vi "PicoScope3000aExampleStreamingMSO.vi"() -> ()   [LabVIEW 2010]
doc: "This example demonstrates how to use the PicoScope Labview library to stream data from a PicoScope 5000 Series Device"
uses:
  ps3000a.dll
  ps3000aWrap.dll
  <vilib>/Waveform/DWDTOps.llb/DWDT Analog to Digital.vi
  PicoScope3000aLib/PicoScope3000aAnalogChannelSettings.ctl
  PicoScope3000aLib/PicoScope3000aDigitalChannelSettings.ctl
panel:
  in  "Port 0 Settings":T1={"Enabled"=FALSE, "Logic Level"=9830} {"Logic Level" items=["1.5V TTL"=9830, "2.5V CMOS"=16383]}
  in  "Trigger Settings":T2={"Trigger Enabled"=FALSE, "Trigger Source"=enum."Channel A", "Trigger Threshold (volts)"=0.0, "Trigger Direction"=2, "Trigger Delay (samples)"=0, "Auto Trigger Time (ms)"=1000} {"Trigger Direction" items=["Above", "Below", "Rising", "Falling", "Rising or Falling"]}
  in  "Channel A Settings":T3={"Enabled"=TRUE, "Coupling"=1, "Range"=6, "Analogue Offset"=0.0, "Bandwidth Limit"=0} {"Bandwidth Limit" items=["Full", "20MHz"]; "Range" items=["10 mV", "20 mV", "50 mV", "100 mV", "200 mV", "500 mV", "1 V", "2 V", "5 V", "10 V", "20 V", "50 V ", "100 V"]; "Coupling" items=["AC", "DC"]}
  out "Analog Channels":T4(graph)
  out "Raw Sample Interval (sec)":dbl=1.0000000130088963e-06 format="%#.5p"
  out "Max ADC value":i16
  out "Chunk time":u32
  out "Elapsed time":dbl
  in  "Poll time (ms)":u32=10 min=1 max=1000 step=1
  in  "Data file":path=path "PicoScope3000aExampleStreaming ChA Data"
  out "size(s)":i32
  out "Queue depth":i32(graph)
  out "queue depth":i32
  in  "Buffer and Transfer Settings":T5={"startIndex"=0, "Samples"=1000000, "Down Sample Ratio"=1, "Down-Sample Mode"=0} {"Down-Sample Mode" items=["None"=0, "Aggregate"=1, "Decimate"=2, "Average"=4]; "Down Sample Ratio" step=1; "Samples" format="%_6p"}
  out "USB Powered":bool=TRUE
  out "USB 3.0 device on non-USB 3.0 Port":bool=TRUE
  out "TriggeredAt (In Buffer)":u32 format="%#.6p"
  out "TriggeredAt (Total samples)":u32 format="%#.6p"
  in  "Acquisition Settings":T6={"Auto Stop"=TRUE, "Desired Sample Interval"=1, "Pre-trigger Samples"=0, "Post-trigger Samples"=1000000, "Down-Sample Ratio"=1, "Down-Sample Mode"=0, "Time Units"=3} {"Time Units" items=["Nanoseconds (ns)"=2, "Microseconds (us)"=3, "Milliseconds (ms)"=4, "Seconds (s)"=5]; "Down-Sample Mode" items=["None"=0, "Aggregate"=1, "Decimate"=2, "Average"=4]; "Post-trigger Samples" format="%#.6p"; "Pre-trigger Samples" format="%#_6p"}
  out "Port 0":digitalwaveform(graph)={"t0"=timestamp(0 s since 1904-01-01), "dt"=1.0000000130088963e-06, "Y"={"transitions"=[], "data"=[]}}
  out "Triggered":bool
  out "DownSample Interval (sec)":dbl=1.0000000130088963e-06 format="%#.5p"
  out "Total Samples":u32 format="%#.6p"
  out "Auto Stopped":bool
  in  "Serial Number":string
  in  "Open Using Serial Number":bool
  out "Number of Samples per Capture":u32 format="%#.6p"
  in  "Apply  Settings":bool
  in  "stop":bool
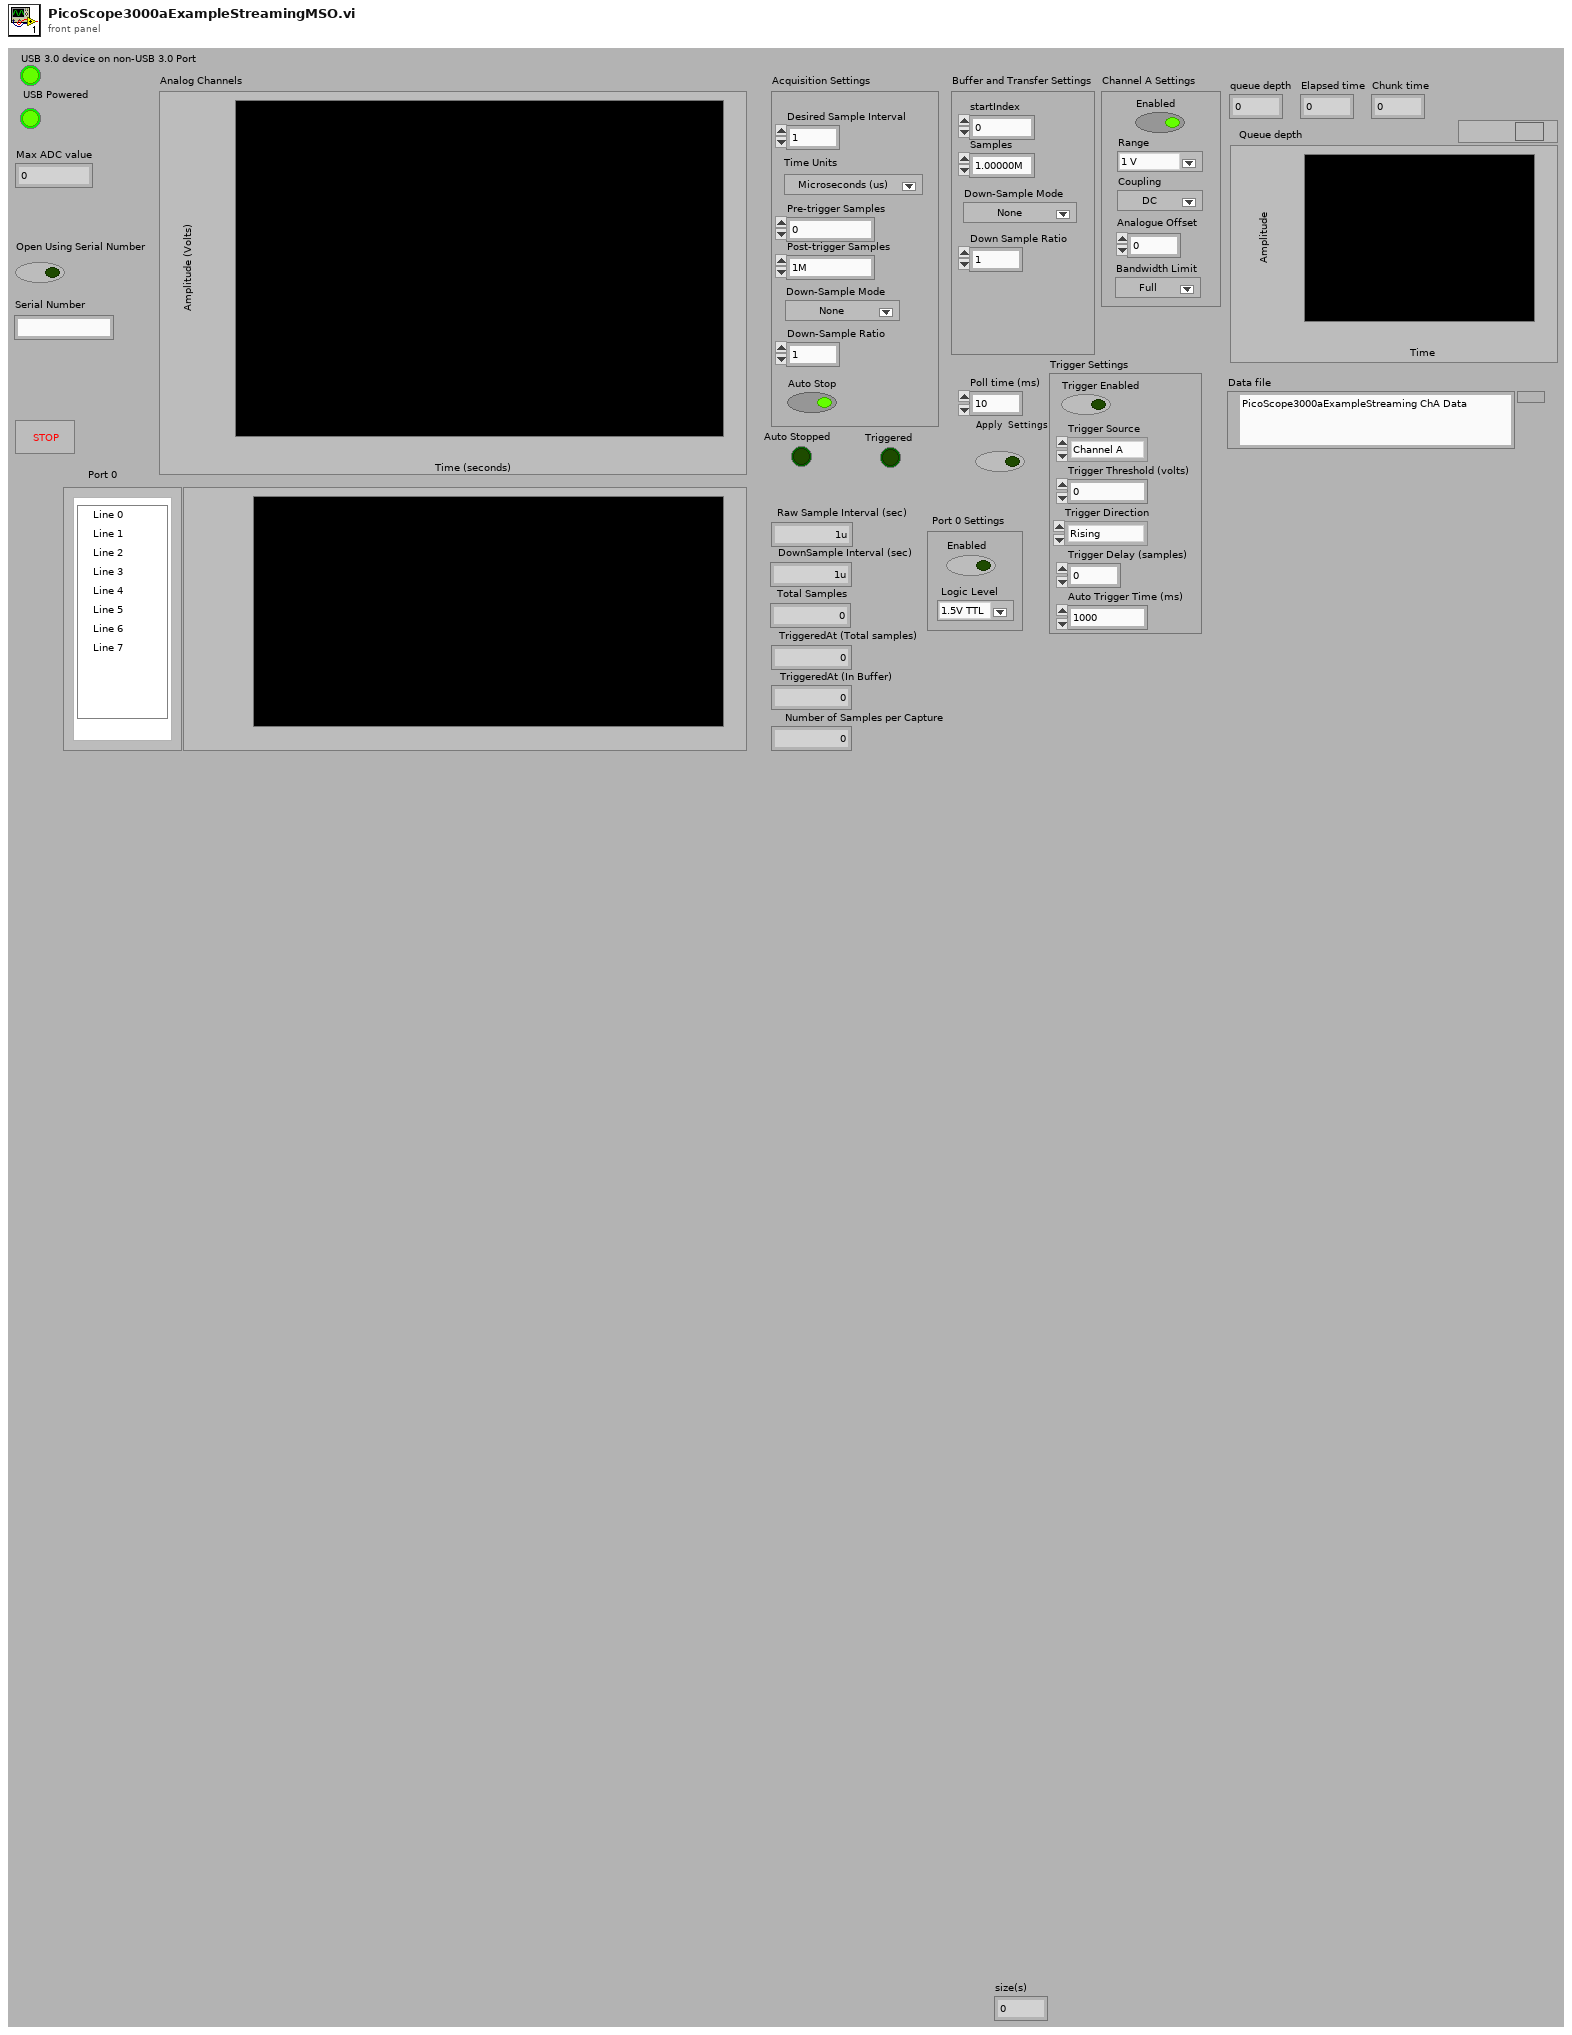
[diagram p1: front panel]
types:
  T1 = typedef "PicoScope3000aDigitalChannelSettings.ctl" = cluster{"Enabled":bool, "Logic Level":i16}
  T2 = cluster{"Trigger Enabled":bool, "Trigger Source":enum32{"Channel A", "Channel B", "Channel C", "Channel D", "Ext."}, "Trigger Threshold (volts)":dbl, "Trigger Direction":u32, "Trigger Delay (samples)":u32, "Auto Trigger Time (ms)":i16}
  T3 = typedef "PicoScope3000aAnalogChannelSettings.ctl" = cluster{"Enabled":bool, "Coupling":u32, "Range":u32, "Analogue Offset":sgl, "Bandwidth Limit":u32}
  T4 = cluster{i32, "DownSample Interval (sec)":dbl, "Data":dbl[]}
  T5 = cluster{"startIndex":u64, "Samples":u64, "Down Sample Ratio":u64, "Down-Sample Mode":u32}
  T6 = cluster{"Auto Stop":bool, "Desired Sample Interval":u32, "Pre-trigger Samples":u32, "Post-trigger Samples":u32, "Down-Sample Ratio":u32, "Down-Sample Mode":i32, "Time Units":u32}
  T7 = enum16{"open", "open or create", "create or replace", "create", "open (read-only)"}
  T8 = cluster{"Driver Version":string, "USB Version":string, "Hardware":string, "Variant":string, "Batch and Serial":string, "Cal Date":string, "Kernel Version":string, "Digital HW Version":string, "Analogue HW Version":string, "MSO":bool, "Number of channels":i16}
  T9 = cluster{"Channel A Buffer":i16[], "Channel B Buffer":i16[], "Channel C Buffer":i16[], "Channel D Buffer":i16[], "Channel E Buffer":i16[], "Channel F Buffer":i16[], "Channel G Buffer":i16[], "Channel H Buffer":i16[], "Port 0":i16[], "Port 1":i16[]}
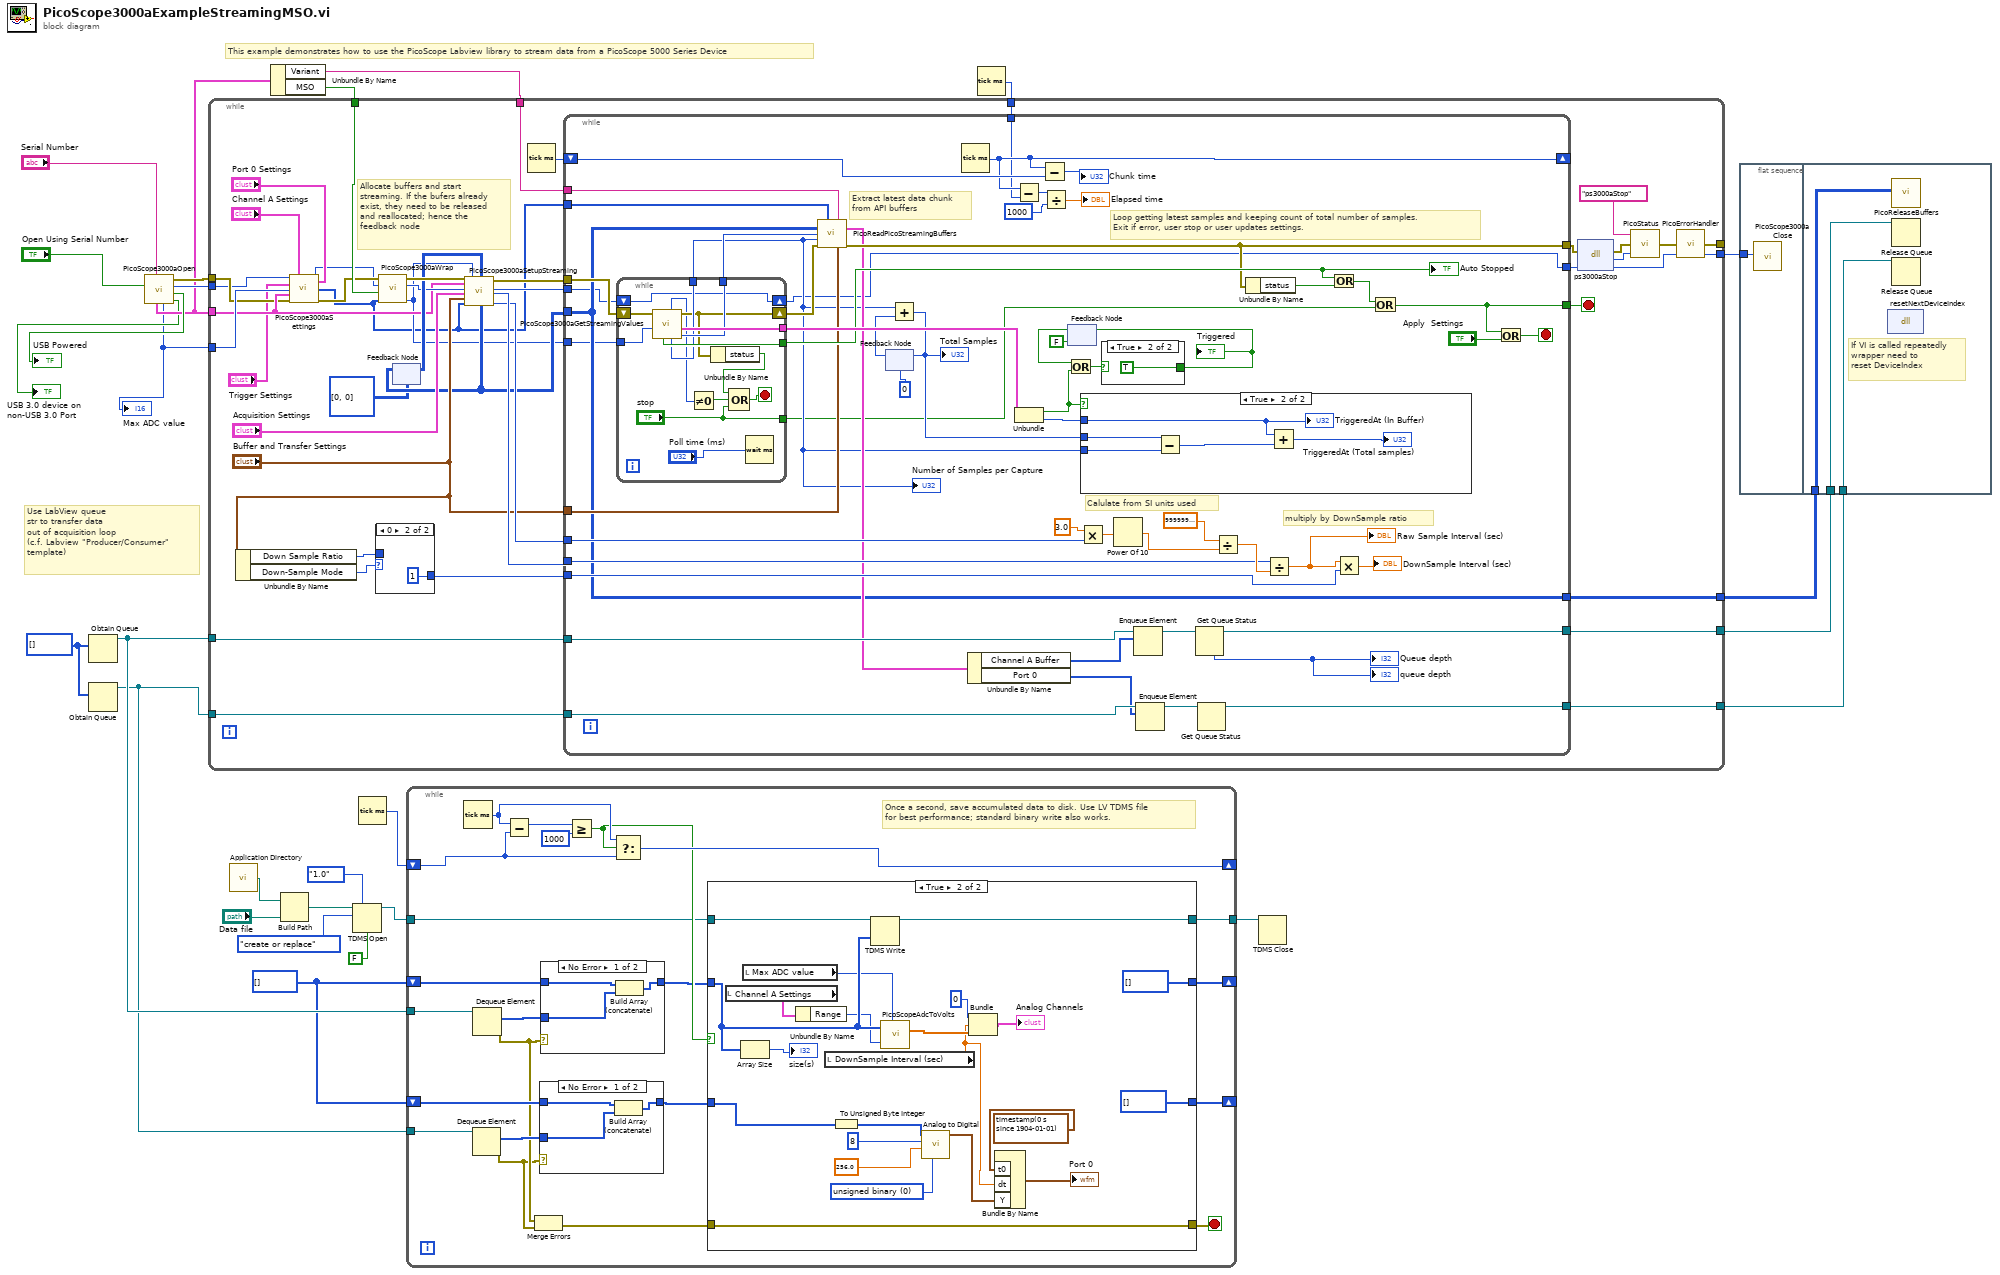
[diagram p0: block diagram]
diagram:
  w9 = i16[] [] ("History Data")
  w12 = i16[] [] ("History Data")
  # "Use LabView queue\nstr to transfer data\nout of acquisition loop\n(c.f. Labview \"Producer/Consumer\"\ntemplate)"
  # "This example demonstrates how to use the PicoScope Labview library to stream data from a PicoScope 5000 Series Device"
  n1 = Obtain Queue(element data type=w12) -> (queue out=w24:refnum<queue>)  [unwired: 4 in, 2 out]
  n2 = Obtain Queue(element data type=w12) -> (queue out=w10:refnum<queue>)  [unwired: 4 in, 2 out]
  n3 = call "PicoScope3000aOpen.vi"("Batch/Serial"="Serial Number", "Use Serial number"="Open Using Serial Number") -> ("USB 3.0 device on non-USB 3.0 Port"=→"USB 3.0 device on non-USB 3.0 Port":bool, "USB Powered"=→"USB Powered":bool, "handle"=w27:i16, "error out"=w28:errorcluster, "Max ADC value"=w1:i16, "Device Info"=w5:T8)  [unwired: 4 in]
  "Max ADC value" <- w1
  n4 = call <vilib>:"Application Directory.vi"() -> ("Application Directory"=w6:path)
  n5 = Unbundle By Name(w5) -> ("Variant"=w4:string, "MSO"=w3:bool)
  n6 = Build Path(base path=w6, name or relative path="Data file") -> (appended path=w7:path)
  n7 = TDMS Open(6:FALSE ("disable buffering? (T)"), 7:enum16{"1.0", "2.0"}."1.0" ("file format version (2.0)"), 10:T7."create or replace" ("operation (0:open)"), 11:w7) -> (3:w16:refnum<k34>)  [unwired: 2 in, 1 out]
  n8 = Tick Count (ms)() -> (millisecond timer value=w18:u32)
  n9 = while {
    tunnel: w24 -> [w49]
    shift-right: [w40] -> _
    shift-left: w9 -> [w48]
    shift-right: [w43] -> _
    shift-left: w18 -> [w44]
    tunnel: w16 -> [w39]
    tunnel: [w38] -> w15
    tunnel: w10 -> [w36]
    shift-right: [w33] -> _
    shift-left: w9 -> [w35]
    stop <- w29 stop-if-true
    # "Once a second, save accumulated data to disk. Use LV TDMS file\nfor best performance; standard binary write also works."
    n10 = Tick Count (ms)() -> (millisecond timer value=w45:u32)
    n11 = Dequeue Element(queue=w36) -> (element=w37:i16[], error out=w31:errorcluster)  [unwired: 2 in, 2 out]
    n12 = Dequeue Element(queue=w49) -> (element=w50:i16[], error out=w32:errorcluster)  [unwired: 2 in, 2 out]
    n13 = Subtract(x=w45, y=w44) -> (x-y=w47:u32)
    n14 = Merge Errors(w32, w31) -> (w30:errorcluster)
    n15 = case shown="No Error" w31 {
      tunnel: w35 -> [w53 w54]
      tunnel: [w52 w54] -> w34
      tunnel: w37 -> [w51 _]
      frame No Error {
        n16 = Build Array (concatenate)(w53, w51) -> (w52:i16[])
      }
      frame Error {
      }
    }
    n17 = case shown="No Error" w32 {
      tunnel: w48 -> [w83 w84]
      tunnel: [w82 w84] -> w41
      tunnel: w50 -> [w81 _]
      frame No Error {
        n18 = Build Array (concatenate)(w83, w81) -> (w82:i16[])
      }
      frame Error {
      }
    }
    n19 = Greater Or Equal?(x=w47, y=u32 1000) -> (x >= y?=w42:bool)
    n20 = Select(t=w45, s=w42, f=w44) -> (s? t:f=w43:u32)
    n21 = case shown="True" w42 {
      tunnel: w41 -> [w58 w76]
      tunnel: [w58 i16[] [] ("History Data")] -> w40
      tunnel: w39 -> [w57 w78]
      tunnel: [w57 w77] -> w38
      tunnel: w34 -> [w56 w63]
      tunnel: [w56 i16[] [] ("History Data")] -> w33
      tunnel: w30 -> [w55 w59]
      tunnel: [w55 w59] -> w29
      frame False {
      }
      frame True {
        w69 = u16 0 items=["unsigned binary", "offset binary", "2's complement"] ("data format (offset binary)")
        n22 = local read "Channel A Settings"() -> (w60:T3)
        n23 = Array Size(array=w76) -> (size(s)=→"size(s)":i32)
        n24 = local read "Max ADC value"() -> (w72:i16)
        n25 = Unbundle By Name(w60) -> ("Range"=w75:u32)
        n26 = local read "DownSample Interval (sec)"() -> (w64:dbl)
        n27 = To Unsigned Byte Integer(number=w63) -> (unsigned 8bit integer=w68:u8[])
        n28 = TDMS Write(0:w78, 9:w76) -> (4:w77:refnum<k34>)  [unwired: 4 in, 3 out]
        n29 = call "PicoScopeAdcToVolts.vi"("Max_adc"=w72, "Range Index"=w75, "Data"=w76) -> ("Data"=w73:dbl[])
        n30 = call-poly <vilib>:"Analog to Digital.vi"("data format (offset binary)"=w69, "full-scale range (pk-pk)"=256.0, "resolution (16 bit)"=8, "analog waveform"=w68) -> ("digital waveform"=w65:digitalwaveform)  [unwired: 4 in, 3 out]
        n31 = Bundle(0, "DownSample Interval (sec)"=w64, "Data"=w73) -> (→"Analog Channels":T4)  [unwired: 1 in]
        n32 = Bundle By Name("t0"=timestamp(0 s since 1904-01-01), "dt"=w64, "Y"=w65) -> (→"Port 0":digitalwaveform)  [unwired: 1 in]
      }
    }
  }
  n33 = Tick Count (ms)() -> (millisecond timer value=w23:u32)
  n34 = while {
    tunnel: [w123] -> w22
    tunnel: w28 -> [w90]
    tunnel: w27 -> [w89]
    tunnel: w5 -> [w92]
    tunnel: w1 -> [w95]
    tunnel: [w109] -> w20
    tunnel: w24 -> [w108]
    tunnel: [w107] -> w21
    tunnel: [w105] -> _
    tunnel: w23 -> [w103]
    tunnel: [w100] -> w11
    tunnel: w10 -> [w99]
    tunnel: w4 -> [w98]
    tunnel: w3 -> [w96]
    stop <- w127 stop-if-true
    # "Allocate buffers and start\nstreaming. If the bufers already\nexist, they need to be released\nand reallocated; hence the\nfeedback node"
    n35 = Unbundle By Name("Buffer and Transfer Settings") -> ("Down Sample Ratio"=w112:u64, "Down-Sample Mode"=w114:u32)
    n36 = call "PicoScope3000aSettings.vi"("handle in"=w89, "Channel A Settings"="Channel A Settings", "Port 0 Settings"="Port 0 Settings", "Trigger Settings"="Trigger Settings", "Max_adc"=w95, "Device Info"=w92, "error in"=w90) -> ("handle out"=w86:i16, "Enabled Array"=w85:i16[], "error out"=w87:errorcluster)  [unwired: 6 in]
    n37 = case shown="0" w114 {
      tunnel: [w128 u32 1 ("Down-Sample Ratio")] -> w113
      tunnel: w112 -> [w128 _]
      frame Default {
      }
      frame 0 {
      }
    }
    n38 = call "PicoScope3000aWrap.vi"("Enabled Array"=w85, "MSO Device?"=w96, "handle in"=w86, "error in (no error)"=w87) -> ("deviceIndex"=w91:u16, "handle out"=w93:i16, "error out"=w118:errorcluster)  [unwired: 1 in]
    n39 = feedback #1(u64[][] [[0], [0]] ("Pointer array")) -> (w106:u64[][])
    n40 = call "PicoScope3000aSetupStreaming.vi"("error in"=w118, "Device Info"=w92, "handle in"=w93, "Acquisition Settings"="Acquisition Settings", "Buffer and Transfer Settings"="Buffer and Transfer Settings", "enabled array"=w85, "deviceIndex"=w91, "Pointers In"=w106) -> ("Pointer array"=w102:u64[][], "error out"=w125:errorcluster, "handle out"=w126:i16, "Sample Interval"=w117:u32, "sampleIntervalTimeUnits"=w116:u32)  [unwired: 7 in]
    n41 = feedback-in #1(w102) -> ()
    n42 = Tick Count (ms)() -> (millisecond timer value=w104:u32)
    n43 = while {
      tunnel: [w130] -> w124
      tunnel: [w184] -> w127
      tunnel: w126 -> [w131]
      tunnel: w125 -> [w160]
      tunnel: w117 -> [w163]
      tunnel: w116 -> [w171]
      tunnel: [w157] -> w115
      tunnel: w113 -> [w161]
      tunnel: "Buffer and Transfer Settings" -> [w159]
      tunnel: w85 -> [w156]
      tunnel: [w154] -> w109
      tunnel: w108 -> [w152]
      tunnel: w102 -> [w150]
      tunnel: [w150] -> w107
      shift-right: [w145] -> _
      shift-left: w104 -> [w146]
      tunnel: w103 -> [w144]
      tunnel: w98 -> [w139]
      tunnel: [w136] -> w100
      tunnel: w99 -> [w135]
      tunnel: w91 -> [w132]
      stop <- w183 stop-if-true
      # "Loop getting latest samples and keeping count of total number of samples. \nExit if error, user stop or user updates settings."
      # "Extract latest data chunk\nfrom API buffers"
      # "Calulate from SI units used"
      # "multiply by DownSample ratio"
      n44 = while {
        tunnel: [w199] -> w182
        tunnel: [w198] -> w179
        tunnel: [w196] -> w141
        tunnel: [w195] -> w140
        shift-right: [w187] -> w130
        shift-left: w131 -> [w187]
        shift-right: [w194] -> w158
        shift-left: w160 -> [w197]
        tunnel: ["stop"] -> w133
        tunnel: w132 -> [w186]
        stop <- w189 stop-if-true
        n45 = call "PicoScope3000aGetStreamingValues.vi"("deviceIndex"=w186, "error in"=w197) -> ("Start Index"=w196:u32, "Trigger"=w199:cluster{bool, "triggeredAt (Total samples)":u32}, "error out"=w194:errorcluster, "Number of Samples"=w195:i32, "ready"=w192:i16, "Auto Stopped"=w198:bool)  [unwired: 4 in]
        n46 = Not Equal To 0?(x=w192) -> (x != 0?=w190:bool)
        n47 = Unbundle By Name(w194) -> ("status"=w191:bool)
        n48 = Compound Arithmetic op=OR(w191, w190, "stop") -> (w189:bool)
        n49 = Wait (ms)(milliseconds to wait="Poll time (ms)") -> ()  [unwired: 1 out]
      }
      "Number of Samples per Capture" <- w140
      "Auto Stopped" <- w179
      n50 = call "PicoReadPicoStreamingBuffers.vi"("enabled array"=w156, "Buffer and Transfer Settings"=w159, "Variant"=w139, "Pointer array"=w150, "Offset Index"=w141, "Number of Samples"=w140, "error in (no error)"=w158) -> ("Buffers (Max or non-aggregated)"=w151:T9, "error out"=w157:errorcluster)  [unwired: 6 in, 1 out]
      n51 = feedback #2(u32 0) -> (w175:u32)
      n52 = Add(x=w140, y=w175) -> (x+y=w167:u32)
      "Total Samples" <- w167
      n53 = feedback-in #2(w167) -> ()
      n54 = Tick Count (ms)() -> (millisecond timer value=w145:u32)
      n55 = Unbundle By Name(w151) -> ("Channel A Buffer"=w142:i16[], "Port 0"=w134:i16[])
      n56 = Subtract(x=w145, y=w144) -> (x-y=w149:u32)
      n57 = Unbundle(w182) -> (w165:bool, "triggeredAt (Total samples)"=w164:u32)
      n58 = Subtract(x=w145, y=w146) -> (x-y=→"Chunk time":u32)
      n59 = Divide(x=w149, y=u32 1000) -> (x/y=→"Elapsed time":dbl)
      n60 = feedback #3(FALSE) -> (w177:bool)
      n61 = Or(x=w177, y=w165) -> (x .or. y?=w168:bool)
      n62 = Multiply(x=3.0, y=w171) -> (x*y=w169:dbl)
      n63 = case shown="True" w165 {
        tunnel: w140 -> [_ w200]
        tunnel: w167 -> [_ w204]
        tunnel: w164 -> [_ w202]
        frame False {
        }
        frame True {
          n64 = Subtract(x=w204, y=w200) -> (x-y=w203:u32)
          n65 = Add(x=w202, y=w203) -> (x+y=→"TriggeredAt (Total samples)":u32)
          "TriggeredAt (In Buffer)" <- w202
        }
      }
      n66 = case shown="True" w168 {
        selector: w168 -> [w205 _]
        tunnel: [w205 TRUE] -> w166
        frame False {
        }
        frame True {
        }
      }
      "Triggered" <- w166
      n67 = feedback-in #3(w166) -> ()
      n68 = Power Of 10(x=w169) -> (10^x=w170:dbl)
      n69 = Enqueue Element(queue=w152, element=w142) -> (queue out=w153:refnum<queue>)  [unwired: 2 in, 2 out]
      n70 = Enqueue Element(queue=w135, element=w134) -> (queue out=w137:refnum<queue>)  [unwired: 2 in, 2 out]
      n71 = Get Queue Status(queue=w153) -> (queue out=w154:refnum<queue>, # elements in queue=→"queue depth" →"Queue depth":i32)  [unwired: 2 in, 6 out]
      n72 = Get Queue Status(queue=w137) -> (queue out=w136:refnum<queue>)  [unwired: 2 in, 7 out]
      n73 = Divide(x=sgl 1000000000000000.0 ("y"), y=w170) -> (x/y=w172:dbl)
      n74 = Unbundle By Name(w157) -> ("status"=w181:bool)
      n75 = Divide(x=w163, y=w172) -> (x/y=w138:dbl)
      "Raw Sample Interval (sec)" <- w138
      n76 = Or(x=w179, y=w181) -> (x .or. y?=w180:bool)
      n77 = Multiply(x=w138, y=w161) -> (x*y=→"DownSample Interval (sec)":dbl)
      n78 = Or(x=w180, y=w133) -> (x .or. y?=w184:bool)
      n79 = Or(x=w184, y="Apply  Settings") -> (x .or. y?=w183:bool)
    }
    n80 = dll-call lib="ps3000a.dll" fn="ps3000aStop"(error in=w115, "handle"=w124) -> (error out=w121:errorcluster, "PICO_STATUS"=w122:u32, "handle"=w123:i16)  [unwired: 2 in, 1 out]
    n81 = call "PicoStatus.vi"("PICO STATUS"=w122, "error in"=w121, "source"="ps3000aStop") -> ("error out"=w120:errorcluster)
    n82 = call "PicoErrorHandler.vi"("error in"=w120) -> ("error out"=w105:errorcluster)
  }
  n83 = TDMS Close(11:w15) -> ()  [unwired: 1 in, 2 out]
  n84 = flat-sequence {
    tunnel: w22 -> [w207]
    tunnel: w21 -> [w210]
    tunnel: w20 -> [w209]
    tunnel: w11 -> [w208]
    frame #0 {
      n85 = call "PicoScope3000aClose.vi"("handle"=w207) -> ()
    }
    frame #1 {
      # "If VI is called repeatedly\nwrapper need to\nreset DeviceIndex"
      n86 = dll-call lib="ps3000aWrap.dll" fn="resetNextDeviceIndex"() -> ()  [unwired: 4 in, 2 out]
      n87 = call "PicoReleaseBuffers.vi"("Pointer array"=w210) -> ()  [unwired: 10 in, 1 out]
      n88 = Release Queue(queue=w209) -> ()  [unwired: 2 in, 3 out]
      n89 = Release Queue(queue=w208) -> ()  [unwired: 2 in, 3 out]
    }
  }
